vi "SET_Glyph.vi"(8 "error in":errorcluster, 10 "Coordinates":T5, 11 "Data in":T1={"Class"={"Ants"=refnum, "Layer"=refnum, "Templates"=refnum, "Icon"=refnum, "Glyph"=refnum, "Settings"=refnum, "Tools"=refnum, "History"=refnum}, "Ref"={"Add Layer"=refnum, "Remove Layer"=refnum, "Line Text"=[], "Body Text Spec"=refnum, "DNL_Font"=refnum, "glyph path str"=refnum, "templates path str"=refnum, "Arrow Up"=refnum, "Arrow Down"=refnum, "IE VI Ref"=refnum, "Glyphs tree"=refnum, "Templates tree"=refnum, "Layer Icon Text"=refnum, "Layer Template"=refnum, "Body Text"=refnum, "Search Templates"=refnum, "TextMarker"=refnum, "Tab Control"=refnum, "Search Glyphs"=refnum, "Line Color"=refnum, "DNL_Glyphs []"=refnum, "Fill Color"=refnum, "Tools"=refnum, "Icon"=refnum, "Preview"=refnum, "Ants"=refnum, "Terminals"=refnum, "menu reference"=refnum, "LayerNames"=[], "GlyphLoadAnimation"=refnum, "TemplateLoadAnimation"=refnum, "refreshGlyphs"=refnum, "refreshTemplates"=refnum}, "Support"={"AntsRect"={"left"=0, "top"=0, "right"=0, "bottom"=0}, "Mouse Move Coords"={"Horizontal"=0, "Vertical"=0}, "Mouse Down Coords"={"Horizontal"=0, "Vertical"=0}, "Temp Coord"={"Horizontal"=0, "Vertical"=0}, "Action"=enum."Default", "Edge Color"=4914962, "Fill Color"=16860, "Mouse Down?"=FALSE, "Draft Mode?"=FALSE, "Temp Icon"=bytes[3102], "CTRL Pressed"=FALSE, "Move Selection?"=FALSE, "AntsRect Orig"={"left"=0, "top"=0, "right"=0, "bottom"=0}, "Text"="", "TM Set?"=FALSE, "Mouse inside icon?"=FALSE, "Tool (old value)"=0, "Pencil Move Color"=0, "Swap Colors?"=FALSE, "Shift pressed?"=FALSE}}) -> (0 "error out":errorcluster, 1 "All Layers":refnum<class "Layer.lvclass">[](array[class]), 3 "Data out":T1={"Class"={"Ants"=refnum, "Layer"=refnum, "Templates"=refnum, "Icon"=refnum, "Glyph"=refnum, "Settings"=refnum, "Tools"=refnum, "History"=refnum}, "Ref"={"Add Layer"=refnum, "Remove Layer"=refnum, "Line Text"=[], "Body Text Spec"=refnum, "DNL_Font"=refnum, "glyph path str"=refnum, "templates path str"=refnum, "Arrow Up"=refnum, "Arrow Down"=refnum, "IE VI Ref"=refnum, "Glyphs tree"=refnum, "Templates tree"=refnum, "Layer Icon Text"=refnum, "Layer Template"=refnum, "Body Text"=refnum, "Search Templates"=refnum, "TextMarker"=refnum, "Tab Control"=refnum, "Search Glyphs"=refnum, "Line Color"=refnum, "DNL_Glyphs []"=refnum, "Fill Color"=refnum, "Tools"=refnum, "Icon"=refnum, "Preview"=refnum, "Ants"=refnum, "Terminals"=refnum, "menu reference"=refnum, "LayerNames"=[], "GlyphLoadAnimation"=refnum, "TemplateLoadAnimation"=refnum, "refreshGlyphs"=refnum, "refreshTemplates"=refnum}, "Support"={"AntsRect"={"left"=0, "top"=0, "right"=0, "bottom"=0}, "Mouse Move Coords"={"Horizontal"=0, "Vertical"=0}, "Mouse Down Coords"={"Horizontal"=0, "Vertical"=0}, "Temp Coord"={"Horizontal"=0, "Vertical"=0}, "Action"=enum."Default", "Edge Color"=4914962, "Fill Color"=16860, "Mouse Down?"=FALSE, "Draft Mode?"=FALSE, "Temp Icon"=bytes[3102], "CTRL Pressed"=FALSE, "Move Selection?"=FALSE, "AntsRect Orig"={"left"=0, "top"=0, "right"=0, "bottom"=0}, "Text"="", "TM Set?"=FALSE, "Mouse inside icon?"=FALSE, "Tool (old value)"=0, "Pencil Move Color"=0, "Swap Colors?"=FALSE, "Shift pressed?"=FALSE}})   [LabVIEW 2020]
uses:
  vi.lib/LabVIEW Icon API/lv_icon/Classes/Layer/Layer.lvclass
  Class/Ants/Ants.lvclass
  Class/FakedArray/FakedArray.lvclass
  vi.lib/LabVIEW Icon API/lv_icon/Classes/Icon/Icon.lvclass
  Class/Icon Library/Glyph.lvclass
  Class/Settings/Settings.lvclass
  Class/Tools/Tools Paint.lvclass
  vi.lib/LabVIEW Icon API/lv_icon/Controls/LayerType.ctl
  <vilib>/Utility/miscctls.llb/LVPoint32TypeDef.ctl
  Controls/SupportClass_Action.ctl
  vi.lib/LabVIEW Icon API/lv_icon/Controls/IEColor.ctl
  Controls/Support Cluster.ctl
  lv_icon.lvlib
  Controls/References Cluster.ctl
  Controls/IE Classes.ctl
  Controls/Global Data.ctl
  History/History/History.lvclass
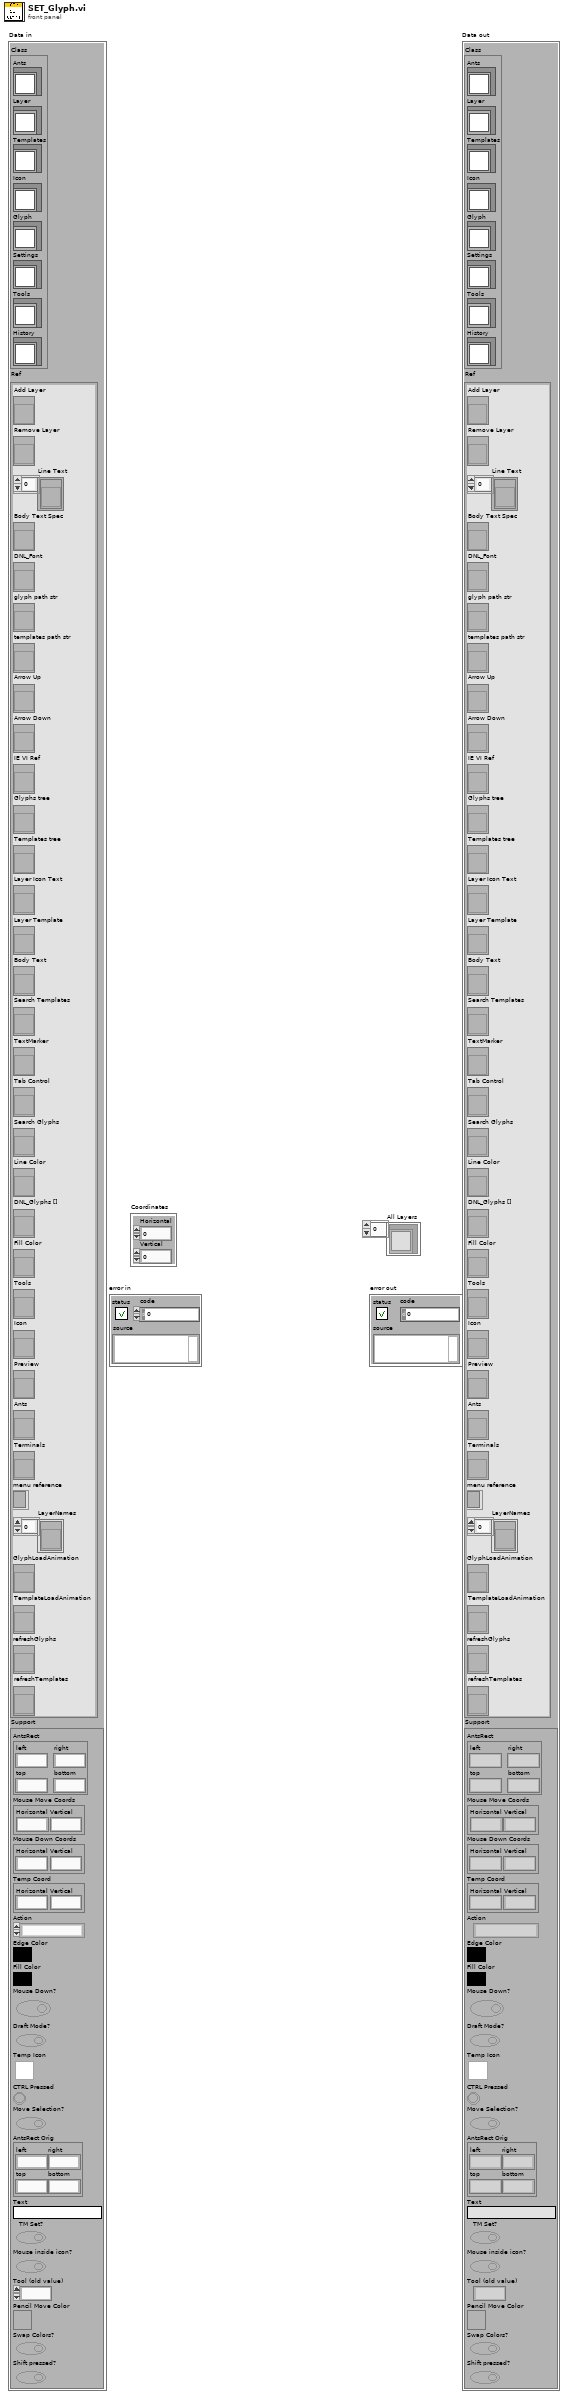
[diagram p1: front panel]
types:
  T1 = typedef "lv_icon.lvlib/Global Data.ctl" = cluster{"Class":T2, "Ref":T3, "Support":T4}
  T2 = typedef "lv_icon.lvlib/IE Classes.ctl" = cluster{"Ants":refnum<class "Ants.lvclass">, "Layer":refnum<class "FakedArray.lvclass">, "Templates":refnum<class "FakedArray.lvclass">, "Icon":refnum<class "Icon.lvclass">, "Glyph":refnum<class "Glyph.lvclass">, "Settings":refnum<class "Settings.lvclass">, "Tools":refnum<class "Tools Paint.lvclass">, "History":refnum<class "History.lvclass">}
  T3 = typedef "lv_icon.lvlib/References Cluster.ctl" = cluster{"Add Layer":refnum<vi>, "Remove Layer":refnum<vi>, "Line Text":refnum<vi>[], "Body Text Spec":refnum<vi>, "DNL_Font":refnum<vi>, "glyph path str":refnum<vi>, "templates path str":refnum<vi>, "Arrow Up":refnum<vi>, "Arrow Down":refnum<vi>, "IE VI Ref":refnum<vi>, "Glyphs tree":refnum<vi>, "Templates tree":refnum<vi>, "Layer Icon Text":refnum<vi>, "Layer Template":refnum<vi>, "Body Text":refnum<vi>, "Search Templates":refnum<vi>, "TextMarker":refnum<vi>, "Tab Control":refnum<vi>, "Search Glyphs":refnum<vi>, "Line Color":refnum<vi>, "DNL_Glyphs []":refnum<vi>, "Fill Color":refnum<vi>, "Tools":refnum<vi>, "Icon":refnum<vi>, "Preview":refnum<vi>, "Ants":refnum<vi>, "Terminals":refnum<vi>, "menu reference":refnum<k9>, "LayerNames":refnum<vi>[], "GlyphLoadAnimation":refnum<vi>, "TemplateLoadAnimation":refnum<vi>, "refreshGlyphs":refnum<vi>, "refreshTemplates":refnum<vi>}
  T4 = typedef "lv_icon.lvlib/Support Cluster.ctl" = cluster{"AntsRect":cluster{"left":i16, "top":i16, "right":i16, "bottom":i16}, "Mouse Move Coords":T5, "Mouse Down Coords":T5, "Temp Coord":T5, "Action":T6, "Edge Color":T7, "Fill Color":T7, "Mouse Down?":bool, "Draft Mode?":bool, "Temp Icon":picture, "CTRL Pressed":bool, "Move Selection?":bool, "AntsRect Orig":cluster{"left":i16, "top":i16, "right":i16, "bottom":i16}, "Text":string, "TM Set?":bool, "Mouse inside icon?":bool, "Tool (old value)":u32, "Pencil Move Color":u32, "Swap Colors?":bool, "Shift pressed?":bool}
  T5 = typedef "LVPoint32TypeDef.ctl" = cluster{"Horizontal":i32, "Vertical":i32}
  T6 = typedef "SupportClass_Action.ctl" = enum16{"Default", "Move Selection", "Glyph Library", "Tool"}
  T7 = typedef "IEColor.ctl" = u32
  T8 = typedef "LayerType.ctl" = enum16{"Graphic", "Text", "Tool", "Graphic Drop"}
  T9 = typedef "Graphic.ctl" = cluster{"Rectangle":cluster{"left":i16, "top":i16, "right":i16, "bottom":i16}, "Path":path, "Image":picture, "Filter":string, "FileName":string}
  T10 = typedef "lv_icon.lvlib/INI Data.ctl" = cluster{"Show Terminals?":bool, "Text":cluster{"Font":T11, "Alignment":T12, "Size":T13}, "3rd party Templates":cluster{"Store 3rd party Templates?":bool, "Folder Name":string}, "Merge user layers on commit":bool, "Body Text":T14, "Fill Color":T7, "Edge Color":T7, "Tab":u16, "Tool":T15, "Disable Layers?":bool}
  T11 = typedef "Font.ctl" = string
  T12 = typedef "Alignment.ctl" = u16
  T13 = typedef "Font Size.ctl" = u8
  T14 = typedef "BodyText.ctl" = cluster{"Line 1 text":string, "Line 2 text":string, "Line 3 text":string, "Line 4 text":string, "Line 1 color":u32, "Line 2 color":u32, "Line 3 color":u32, "Line 4 color":u32, "Body Text Spec":cluster{"Font":T11, "Alignment":T12, "Size":u8}, "Center text vertically":bool, "Capitalize Text":bool}
  T15 = typedef "Tools.ctl" = enum32{"Pencil", "Line", "Dropper", "Fill", "Rectangle", "Filled Rectangle", "Ellipse", "Filled Ellipse", "Eraser", "Text", "Select", "Move"}
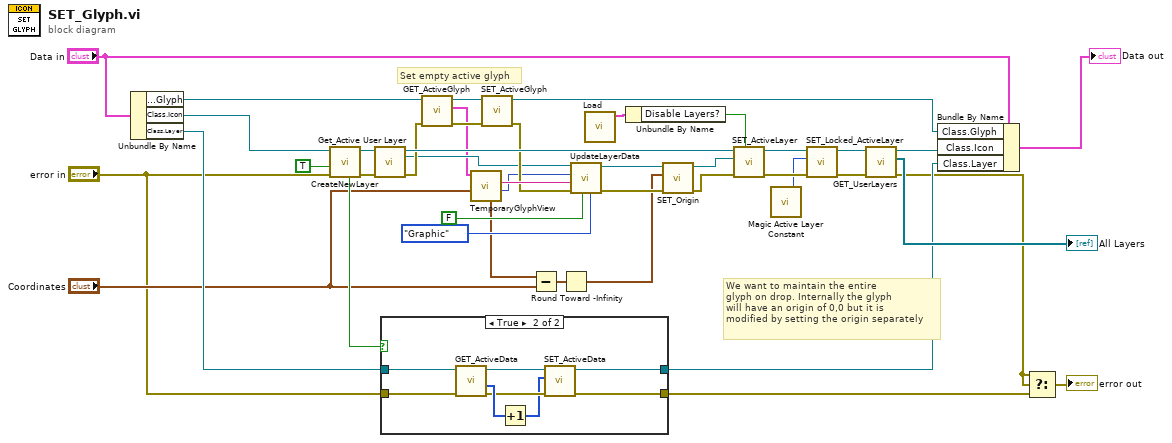
[diagram p0: block diagram]
diagram:
  # "We want to maintain the entire\nglyph on drop. Internally the glyph\nwill have an origin of 0,0 but it is\nmodified by setting the origin separately"
  # "Set empty active glyph"
  n1 = Unbundle By Name("Data in") -> ("Class.Glyph"=w23:refnum<class "Glyph.lvclass">, "Class.Icon"=w22:refnum<class "Icon.lvclass">, "Class.Layer"=w18:refnum<class "FakedArray.lvclass">)
  n2 = call "CreateNewLayer.vi"("error in"="error in", "Force New Layer?"=TRUE, "Icon.lvclass"=w22) -> ("error out"=w34:errorcluster, "Icon.lvclass out"=w33:refnum<class "Icon.lvclass">, "Layer added?"=w27:bool)  [unwired: 2 in, 4 out]
  n3 = call-dynamic "Get_Active User Layer.vi"("error in (no error)"=w34, "Icon in"=w33) -> ("error out"=w36:errorcluster, "Layer.lvclass"=w35:refnum<class "Layer.lvclass">, "Icon out"=w40:refnum<class "Icon.lvclass">)  [unwired: 7 out]
  n4 = case shown="True" w27 {
    tunnel: "error in" -> [w45 w46]
    tunnel: [w45 w47] -> w26
    tunnel: w18 -> [w44 w49]
    tunnel: [w44 w48] -> w17
    frame False {
    }
    frame True {
      n5 = call-dynamic "GET_ActiveData.vi"("error in (no error)"=w46, "FakedArray in"=w49) -> ("error out"=w51:errorcluster, "Active Data []"=w52:i32[], "FakedArray out"=w53:refnum<class "FakedArray.lvclass">)  [unwired: 7 out]
      n6 = Increment(x=w52) -> (x+1=w50:i32[])
      n7 = call-dynamic "SET_ActiveData.vi"("error in (no error)"=w51, "Active Data"=w50, "FakedArray.lvclass in"=w53) -> ("error out"=w47:errorcluster, "FakedArray.lvclass out"=w48:refnum<class "FakedArray.lvclass">)  [unwired: 7 out]
    }
  }
  n8 = call-dynamic "GET_ActiveGlyph.vi"("error in (no error)"=w36, "Glyph.lvclass in"=w23) -> ("error out"=w38:errorcluster, "Path & Icon"=w16:T9, "Glyph.lvclass out"=w37:refnum<class "Glyph.lvclass">)  [unwired: 7 out]
  n9 = call "TemporaryGlyphView.vi"("Mouse Coords Pic"="Coordinates", "Path & Icon"=w16) -> ("origin"=w5:picture, "FileName"=w41:string, "Offset"=w6:cluster{"right":dbl, "bottom":dbl})  [unwired: 7 out]
  n10 = call-dynamic "SET_ActiveGlyph.vi"("error in (no error)"=w38, "Glyph in"=w37) -> ("error out"=w39:errorcluster, "Glyph out"=w19:refnum<class "Glyph.lvclass">)  [unwired: 1 in, 7 out]
  n11 = Subtract(x=w6, y="Coordinates") -> (x-y=w9:cluster{dbl, dbl})
  n12 = Round Toward -Infinity(1:w9) -> (0:w7:cluster{dbl, dbl})
  n13 = call "UpdateLayerData.vi"("Type"=LayerType."Graphic", "Overwrite?"=FALSE, "error in"=w39, "LayerName"=w41, "new picture"=w5, "Active Layer"=w35) -> ("error out"=w12:errorcluster, "Layer.lvclass out"=w13:refnum<class "Layer.lvclass">)  [unwired: 2 in, 2 out]
  n14 = call "Load.vi"() -> ("INI Data"=w2:T10)  [unwired: 3 in, 8 out]
  n15 = Unbundle By Name(w2) -> ("Disable Layers?"=w1:bool)
  n16 = call-dynamic "SET_Origin.vi"("error in"=w12, "Point32"=w7, "Layer.lvclass in"=w13) -> ("error out"=w10:errorcluster, "Layer.lvclass out"=w11:refnum<class "Layer.lvclass">)  [unwired: 7 out]
  n17 = call-dynamic "SET_ActiveLayer.vi"("Combine User Layers?"=w1, "error in (no error)"=w10, "Layer.lvclass"=w11, "Icon.lvclass in"=w40) -> ("error out"=w32:errorcluster, "Icon.lvclass out"=w29:refnum<class "Icon.lvclass">)  [unwired: 6 out]
  n18 = call "Magic Active Layer Constant.vi"() -> ("Magic Constant"=w24:i32)  [unwired: 19 out]
  n19 = call-dynamic "SET_Locked_ActiveLayer.vi"("error in (no error)"=w32, "Active Layer"=w24, "Icon.lvclass in"=w29) -> ("error out"=w31:errorcluster, "Icon.lvclass out"=w30:refnum<class "Icon.lvclass">)  [unwired: 1 in, 6 out]
  n20 = call-dynamic "GET_UserLayers.vi"("error in (no error)"=w31, "Icon.lvclass in"=w30) -> ("error out"=w15:errorcluster, "All Layers"=→"All Layers":refnum<class "Layer.lvclass">[], "Icon.lvclass out"=w20:refnum<class "Icon.lvclass">)  [unwired: 7 out]
  n21 = Bundle By Name(cluster="Data in", "Class.Glyph"=w19, "Class.Icon"=w20, "Class.Layer"=w17) -> (→"Data out":T1)
  n22 = Select(t=w15, s=w15, f=w26) -> (s? t:f=→"error out":errorcluster)
